vi "credentials-separated.vi"() -> ()   [LabVIEW 2024]
doc: "Binary-format test sample. Echo returns Notes."
panel:
  out "Echo":string
  in  "Count":i32=42
  in  "Notes":string="WLMARK-connstr Server=db;Pwd=Sup3rS3cret;"
  in  "Settings":cluster{"API Key":string}={"API Key"="WLMARK-apikey-0042"}
  in  "DB Password":string="WLMARK-hunter22-pw"
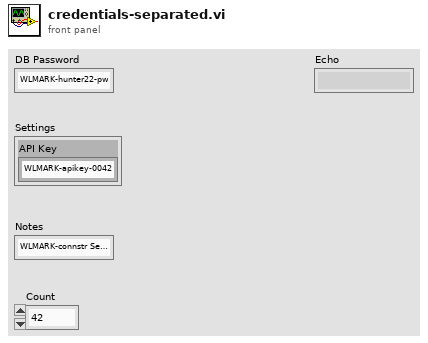
[diagram p1: front panel]
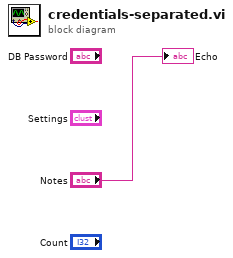
[diagram p0: block diagram]
diagram:
  "Echo" <- "Notes"
